vi "Read thickness from DB.vi"(8 "error in (no error)":errorcluster, 10 "Module?":bool, 11 "Database Entry in":refnum<class "Database Entry.lvclass">) -> (0 "error out":errorcluster, 1 "Baselayer IDs":string[](array[string]), 2 "DB out":string[][](array[string]), 3 "Database Entry out":refnum<class "Database Entry.lvclass">, 5 "Stack names":string[](array[string]))   [LabVIEW 2021, in "Database Entry.lvclass"]
uses:
  Database Entry.lvclass
  Database Entry.lvclass/Database Entry.ctl
  <vilib>/Utility/file.llb/Read Delimited Spreadsheet (string).vi
  Components/Stack/Stack.lvclass
panel:
  out "error out py":errorcluster
  in  "error in (no error) py":errorcluster
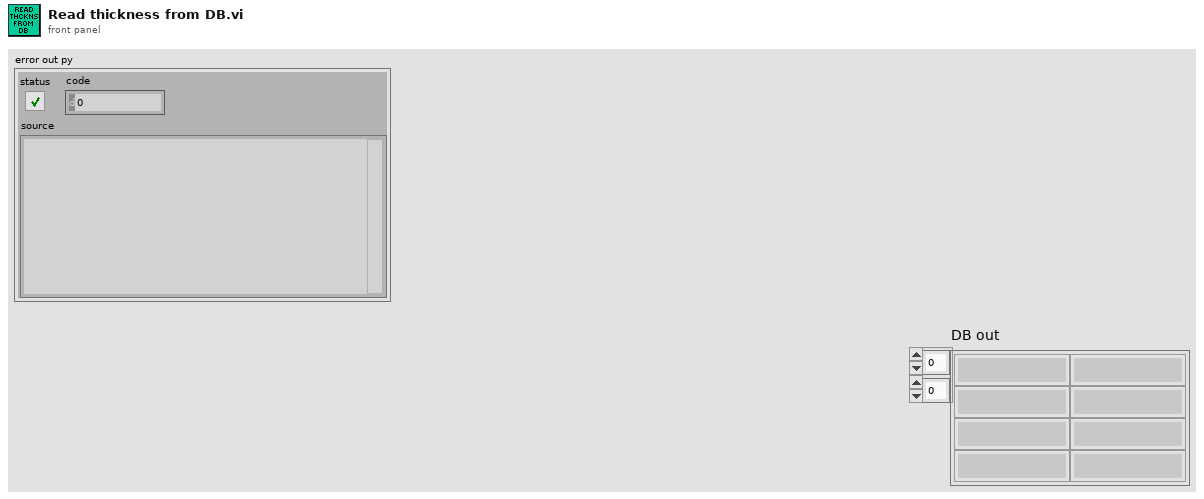
[diagram p1: front panel]
types:
  T1 = cluster{"type (proto/module)":string, " geometry":string, "resolution":string, "baselayer":string, "toplayer":string, "bl_pos":string, "tl_pos":string, "put_pos":string, "region":string, "asstray":string, "comptray":string, "put":string, "date":string, "timestart":string, "timeend":string, "operator":string, "tape":string, "glue":string, "stack name":string, "Adhesive type":string, "Comments":string, "Temperature":string, "Relative Humidity":string}
  T2 = typedef "File Paths.ctl" = cluster{"Glue Pattern Folder":path, "Carrier Tray Folder":path, "Pick Up Tool Fixture Folder":path, "Components Folder":path, "Bellows Tool Offset.txt":path, "Pick Up Tool Offset.txt":path, "Dispense Tip Offset.txt":path, "Log Files":path, "Gantry Assembly Map.txt":path, "Syringe and offset map.txt":path, "Controllers Folder":path, "Local dbase config":path}
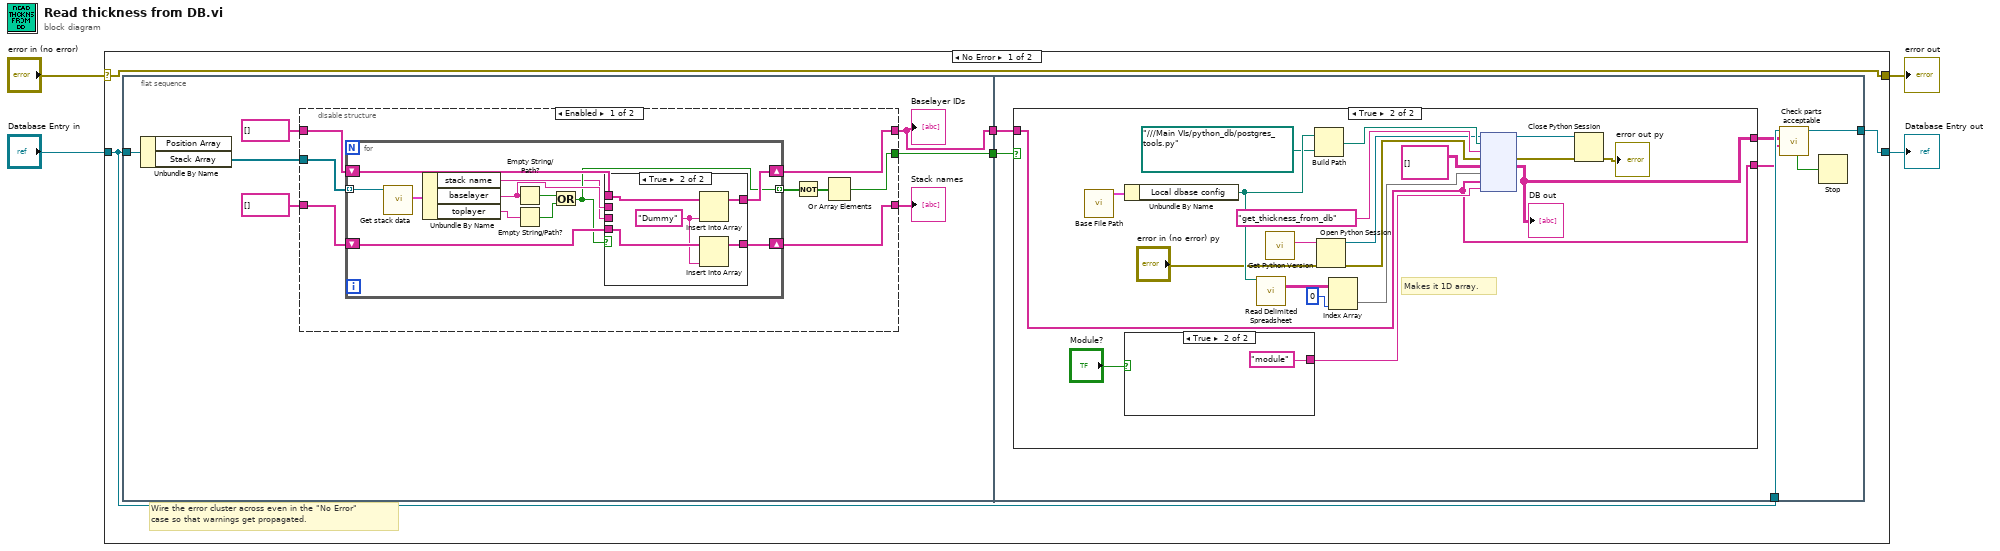
[diagram p0: block diagram]
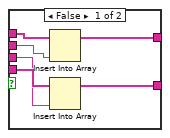
[diagram p2: hidden frame]
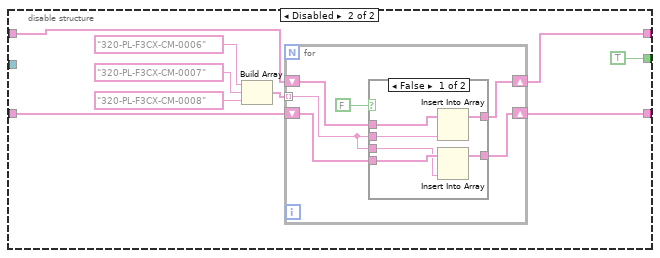
[diagram p3: hidden frame]
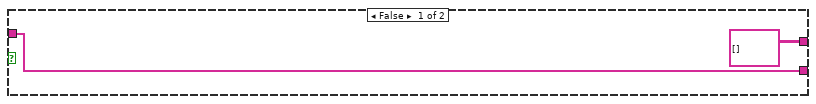
[diagram p5: hidden frame]
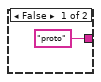
[diagram p6: hidden frame]
diagram:
  n1 = case shown="No Error" "error in (no error)" {
    selector: "error in (no error)" -> [w9 w103]
    tunnel: [w9 w103] -> w3
    tunnel: [w5 w102] -> w1
    tunnel: "Database Entry in" -> [w6 w102]
    frame No Error {
      # "Wire the error cluster across even in the \"No Error\"\ncase so that warnings get propagated."
      n2 = flat-sequence {
        tunnel: [w14] -> w8
        tunnel: [w10] -> w7
        tunnel: w6 -> [w16]
        tunnel: w8 -> [w77]
        tunnel: w7 -> [w76]
        tunnel: w6 -> [w75]
        tunnel: [w73] -> w5
        frame #0 {
          n3 = Unbundle By Name(w16) -> ("Stack Array"=w15:refnum<class "Stack.lvclass">[])  [unwired: 1 out]
          n4 = disable-structure shown="Enabled" {
            disable-tunnel: w15 -> [w24 _]
            disable-tunnel: [w23 w56] -> w14
            disable-tunnel: string[] [] -> [w22 w54]
            disable-tunnel: string[] [] -> [w21 w53]
            disable-tunnel: [w20 w55] -> w11
            disable-tunnel: [w19 TRUE] -> w10
            frame Enabled {
              n5 = for {
                tunnel: w24 -> [w36] mode=indexing
                shift-right: [w30] -> w23
                shift-left: w22 -> [w31]
                shift-right: [w27] -> w20
                shift-left: w21 -> [w28]
                tunnel: [w26] -> w18 mode=indexing
                n6 = call "Get stack data.vi"("Stack in"=w36) -> ("Data cluster"=w33:T1)  [unwired: 8 in, 2 out]
                n7 = Unbundle By Name(w33) -> ("stack name"=w25:string, "baselayer"=w29:string, "toplayer"=w32:string)
                n8 = Empty String/Path?(string/path=w29) -> (empty?=w35:bool)
                n9 = Empty String/Path?(string/path=w32) -> (empty?=w34:bool)
                n10 = Or(x=w35, y=w34) -> (x .or. y?=w26:bool)
                n11 = case shown="True" w26 {
                  tunnel: w31 -> [w42 w47]
                  tunnel: [w41 w46] -> w30
                  tunnel: w29 -> [w40 _]
                  tunnel: w28 -> [w39 w45]
                  tunnel: [w38 w44] -> w27
                  tunnel: w25 -> [w37 _]
                  frame False {
                    n12 = Insert Into Array(array=w42, new element=w40) -> (w41:string[])  [unwired: 1 in]
                    n13 = Insert Into Array(array=w39, new element=w37) -> (w38:string[])  [unwired: 1 in]
                  }
                  frame True {
                    w43 = "Dummy" ("new element/subarray")
                    n14 = Insert Into Array(array=w47, new element=w43) -> (w46:string[])  [unwired: 1 in]
                    n15 = Insert Into Array(array=w45, new element=w43) -> (w44:string[])  [unwired: 1 in]
                  }
                }
              }
              n16 = Not(x=w18) -> (.not. x?=w17:bool[])
              n17 = Or Array Elements(Boolean array=w17) -> (logical OR=w19:bool)
            }
            frame Disabled {
              n18 = Build Array("320-PL-F3CX-CM-0006", "320-PL-F3CX-CM-0007", "320-PL-F3CX-CM-0008") -> (w48:string[])
              n19 = for {
                shift-right: [w62] -> w55
                shift-left: w53 -> [w57]
                shift-right: [w61] -> w56
                shift-left: w54 -> [w58]
                tunnel: w48 -> [w59] mode=indexing
                n20 = case shown="False" FALSE {
                  tunnel: w57 -> [w68 w70]
                  tunnel: [w67 w70] -> w62
                  tunnel: w59 -> [w66 _]
                  tunnel: w58 -> [w65 w69]
                  tunnel: w59 -> [w64 _]
                  tunnel: [w63 w69] -> w61
                  frame False {
                    n21 = Insert Into Array(array=w65, new element=w64) -> (w63:string[])  [unwired: 1 in]
                    n22 = Insert Into Array(array=w68, new element=w66) -> (w67:string[])  [unwired: 1 in]
                  }
                  frame True {
                  }
                }
              }
            }
          }
          "Baselayer IDs" <- w14
          "Stack names" <- w11
        }
        frame #1 {
          n23 = case shown="True" w76 {
            tunnel: w77 -> [w79 w80]
            tunnel: [string[][] [] w81] -> w74
            tunnel: [w79 w80] -> w72
            frame False {
            }
            frame True {
              # "Makes it 1D array."
              n24 = call "Base File Path.vi"() -> ("Paths Out"=w91:T2)  [unwired: 11 in]
              n25 = Unbundle By Name(w91) -> ("Local dbase config"=w94:path)
              n26 = case shown="True" "Module?" {
                tunnel: ["proto" "module"] -> w86
                frame False {
                }
                frame True {
                }
              }
              n27 = call-poly <vilib>:"Read Delimited Spreadsheet.vi"("file path (dialog if empty)"=w94) -> ("all rows"=w90:string[][])  [unwired: 9 in, 5 out]
              n28 = call "Get Python Version.vi"() -> ("Python Version"=w89:string)  [unwired: 10 in, 1 out]
              n29 = Build Path(base path=w94, name or relative path=path "../../../Main VIs/python_db/postgres_tools.py" ("module path")) -> (appended path=w84:path)
              n30 = Open Python Session(python version=w89, 3:"error in (no error) py") -> (session out=w83:refnum<k35>, error out=w82:errorcluster)  [unwired: 1 in]
              n31 = Index Array(array=w90, index (col)=0 ("disabled index (col)")) -> (element=w85:string[])  [unwired: 1 in]
              n32 = node(w83, w84, "get_thickness_from_db" ("function name"), w82, string[][] [], w85, w80, w86) -> (w97:refnum<k35>, w96:errorcluster, w81:string[][])  [unwired: 3 in, 2 out]
              "DB out" <- w81
              n33 = Close Python Session(session in=w97, error in=w96) -> (11:→"error out py":errorcluster)
            }
          }
          n34 = call "Check parts acceptable.vi"("Baselayer IDs"=w72, "DB out"=w74, "Database Entry in"=w75) -> ("Database Entry out"=w73:refnum<class "Database Entry.lvclass">, "Abort?"=w71:bool)  [unwired: 5 in, 2 out]
          n35 = Stop(stop? (T)=w71) -> ()
        }
      }
    }
    frame Error {
    }
  }
  "error out" <- w3
  "Database Entry out" <- w1
